vi "Get Library.vi"(7 "error if not found":bool=TRUE, 8 "error in (no error)":errorcluster, 10 "library name":string, 11 "project ref":refnum<vi>) -> (0 "error out":errorcluster, 1 "found":bool, 2 "library item":refnum<vi>, 3 "project ref out":refnum<vi>)   [LabVIEW 2021, in "MeasurementService Editor.lvlib"]
uses:
  MeasurementService Editor.lvlib
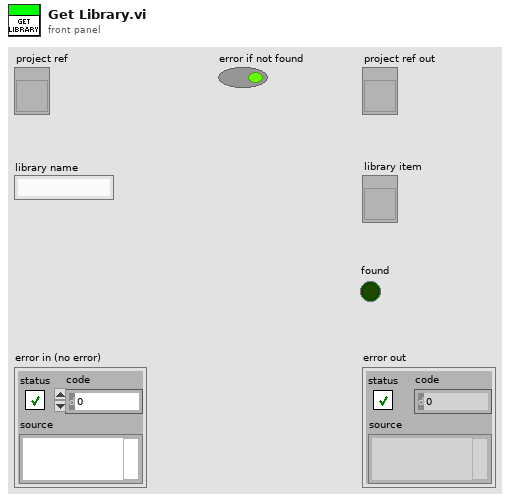
[diagram p1: front panel]
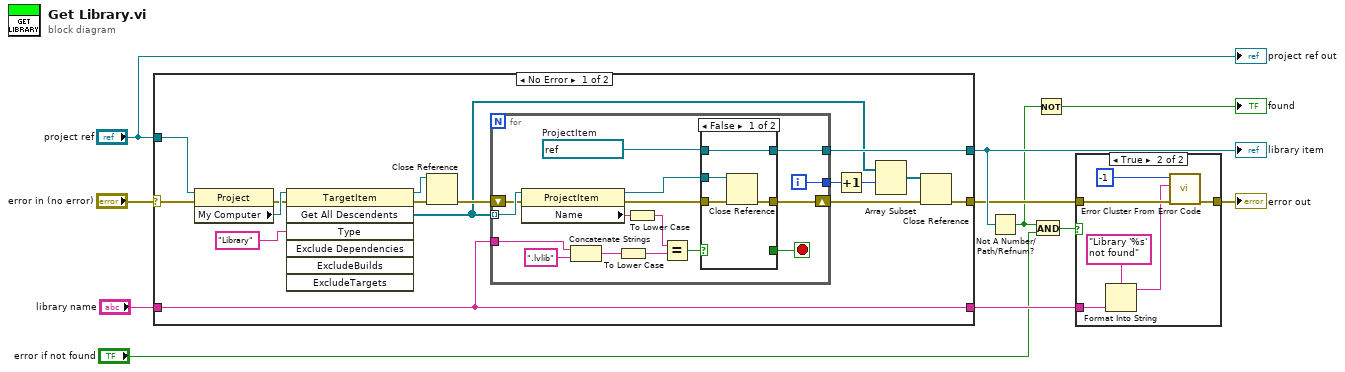
[diagram p0: block diagram]
diagram:
  n1 = case shown="No Error" "error in (no error)" {
    selector: "error in (no error)" -> [w24 w52]
    tunnel: "project ref" -> [w27 _]
    tunnel: "library name" -> [w17 w51]
    tunnel: [w16 w52] -> w6
    tunnel: [w19 _] -> w8
    tunnel: [w17 w51] -> w5
    frame No Error {
      n2 = property class="Project"(reference=w27, error in=w24) -> (error out=w25:errorcluster, "My Computer"=w26:refnum<vi>)  [unwired: 1 out]
      n3 = invoke class="TargetItem" method="Get All Descendents"(reference=w26, error in=w25, "Type"="Library") -> (reference out=w21:refnum<vi>, error out=w22:errorcluster, "All Descendents"=w14:refnum<vi>[])  [unwired: 4 in, 4 out]
      n4 = Close Reference(reference=w21, error in (no error)=w22) -> (error out=w20:errorcluster)
      n5 = for {
        tunnel: w14 -> [w43] mode=indexing
        tunnel: w17 -> [w42]
        shift-right: [w36] -> w23
        shift-left: w20 -> [w40]
        tunnel: [w35] -> w19
        tunnel: [w28] -> w15
        i -> [w28]
        stop <- w30 stop-if-true
        w29 = refnum<vi> refnum  # ProjectItem
        n6 = property class="ProjectItem"(reference=w43, error in=w40) -> (reference out=w38:refnum<vi>, error out=w39:errorcluster, "Name"=w32:string)
        n7 = Concatenate Strings(w42, ".lvlib" ("string")) -> (w34:string)
        n8 = To Lower Case(string=w34) -> (all lower case string=w33:string)
        n9 = To Lower Case(string=w32) -> (all lower case string=w31:string)
        n10 = Equal?(x=w31, y=w33) -> (x = y?=w37:bool)
        n11 = case shown="False" w37 {
          selector: w37 -> [_ w48]
          tunnel: w39 -> [w47 w50]
          tunnel: w38 -> [w44 w49]
          tunnel: [w46 w50] -> w36
          tunnel: [w45 w49] -> w35
          tunnel: w29 -> [w45 _]
          tunnel: [_ w48] -> w30
          frame False {
            n12 = Close Reference(reference=w44, error in (no error)=w47) -> (error out=w46:errorcluster)
          }
          frame True {
          }
        }
      }
      n13 = Increment(x=w15) -> (x+1=w12:i32)
      n14 = Array Subset(array=w14, index=w12) -> (w13:refnum<vi>[])  [unwired: 1 in]
      n15 = Close Reference(reference=w13, error in (no error)=w23) -> (error out=w16:errorcluster)
    }
    frame Error {
    }
  }
  "library item" <- w8
  n16 = Not A Number/Path/Refnum?(number/path/refnum=w8) -> (NaN/Path/Refnum?=w2:bool)
  n17 = And(x=w2, y="error if not found") -> (x .and. y?=w4:bool)
  n18 = Not(x=w2) -> (.not. x?=→"found":bool)
  n19 = case shown="True" w4 {
    tunnel: [w53 w59] -> w7
    tunnel: w6 -> [w53 w58]
    tunnel: w5 -> [_ w54]
    frame False {
    }
    frame True {
      n20 = Format Into String(format string="Library '%s' not found" ("initial string"), w54) -> (resulting string=w55:string)  [unwired: 2 in, 1 out]
      n21 = call <vilib>:"Error Cluster From Error Code.vi"("error in (no error)"=w58, "error message (\"\")"=w55, "error code (0)"=-1) -> ("error out"=w59:errorcluster)  [unwired: 6 in]
    }
  }
  "error out" <- w7
  "project ref out" <- "project ref"
